vi "Install Libraries.vi"() -> ()   [LabVIEW 2021]
doc: "<b>_______________________________________________________________</b>\n** Author: Juan José Villacorta\n** LabVIEW wrapper for C library <b> wiringPi </b>,\n** https://github.com/WiringPi/WiringPi\n<b>_______________________________________________________________</b>\n\n\n/*\n * Install Helper\n ******************************************************************\n */"
uses:
  <vilib>/net/SSH/Client/OpenSSH/OpenSSH Client.lvclass
  C:/Program Files/National Instruments/LabVIEW 2026/vi.lib/net/SSH/Client/Generic/Generic Client.lvclass
  <vilib>/net/SSH/Client/Generic/Generic Client.lvclass/Generic Client.ctl
  <vilib>/net/SFTP/Session/Session.lvclass
  <vilib>/net/SFTP/NI_SFTP.lvlib
  <vilib>/net/SSH/NI_SSH.lvlib
  <vilib>/net/SFTP/API/Upload File.vi
  <vilib>/Utility/error.llb/DialogType.ctl
  <vilib>/net/SFTP/Connect (OpenSSH).vi
panel:
  in  "Close":bool
  in  "Install":bool
  out "Log":string caption="Error output"
  in  "password":string="raspberrypi"
  in  "User":string="pi"
  in  "Host":string="raspberrypi"
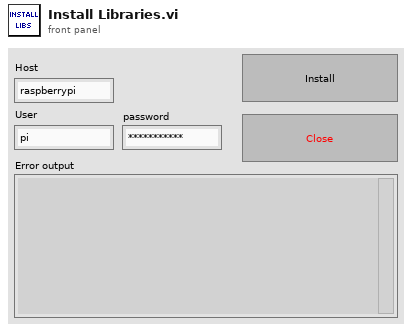
[diagram p1: front panel]
types:
  T1 = typedef "DialogType.ctl" = u16
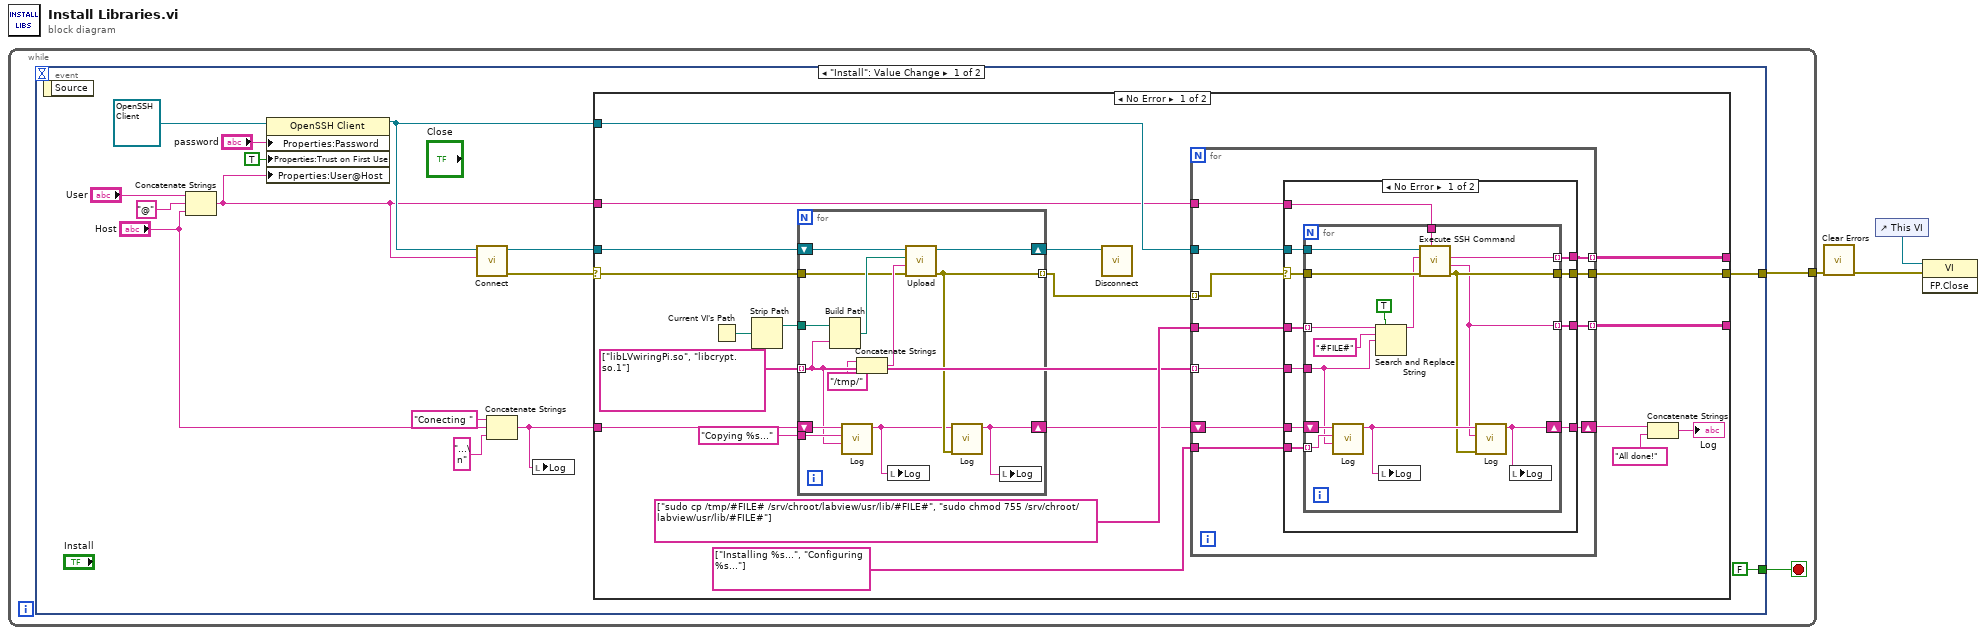
[diagram p0: block diagram]
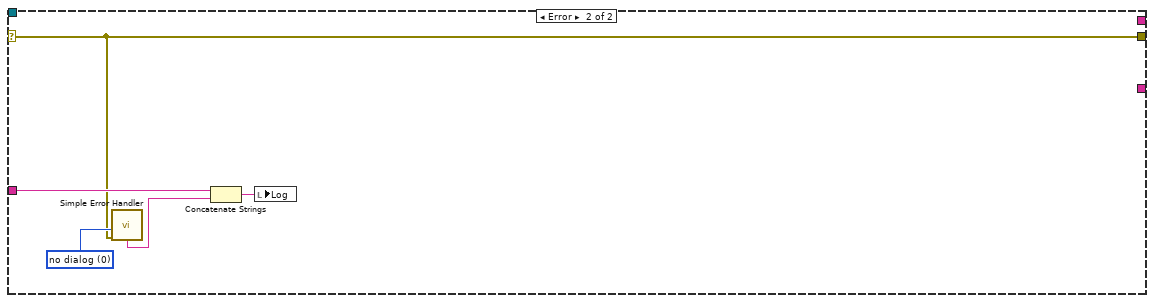
[diagram p3: hidden frame]
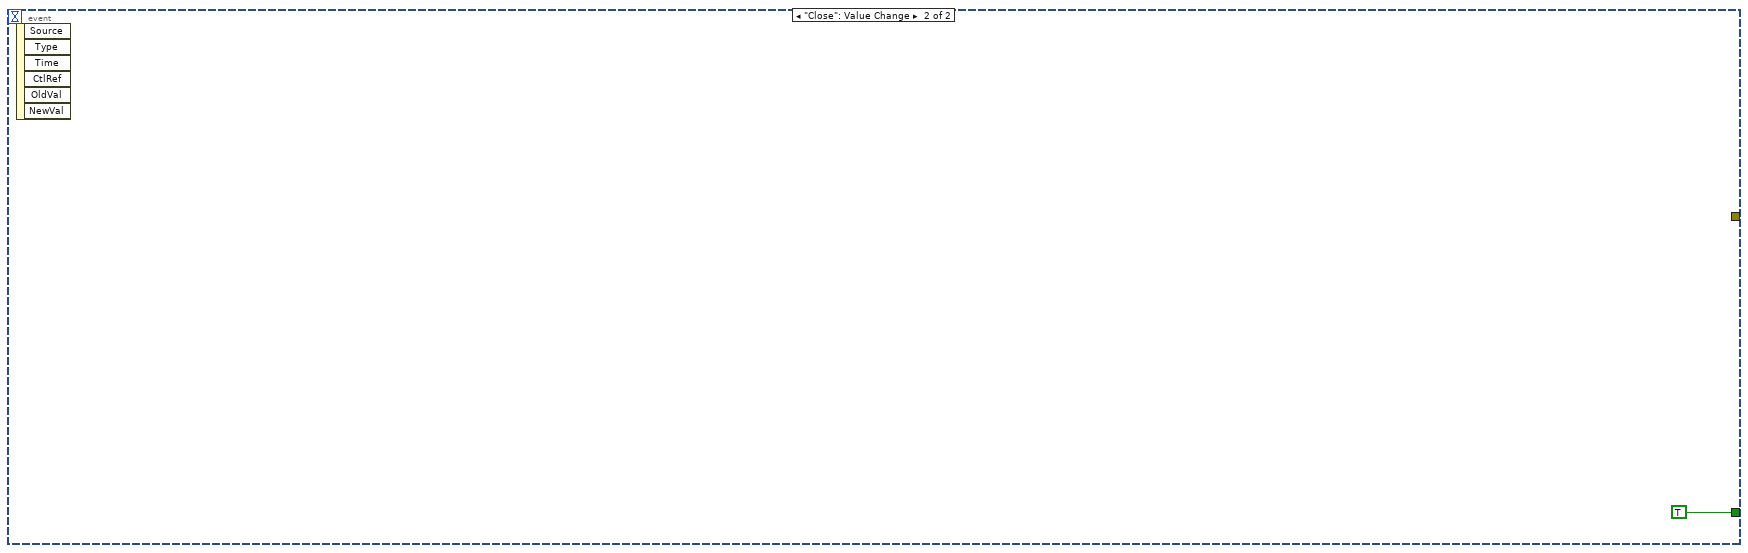
[diagram p4: hidden frame]
diagram:
  n1 = while {
    tunnel: [w5] -> w2
    stop <- w4 stop-if-true
    n2 = event shown="[0] \"Install\": Value Change" {
      selector: _ -> [_ _]
      dyn-events: _ -> [_ _]
      timeout: _ -> [_ _]
      tunnel: [w10 _] -> w5
      tunnel: [FALSE TRUE] -> w4
      event "Install": Value Change {
        n3 = event-data() -> ()  [unwired: 1 in, 1 out]
        n4 = Concatenate Strings("User", "@" ("string"), "Host") -> (w12:string)
        n5 = property class="OpenSSH Client"(reference=refnum<class "OpenSSH Client.lvclass"> refnum ("NI_SSH.lvlib:OpenSSH Client"), "Properties:Password"="password", "Properties:Trust on First Use"=TRUE ("trust on first use"), "Properties:User@Host"=w12) -> (reference out=w13:refnum<class "OpenSSH Client.lvclass">)  [unwired: 1 in, 1 out]
        n6 = call-poly <vilib>:"Connect.vi"("user@host"=w12, "client"=w13) -> ("error out"=w18:errorcluster, "session"=w19:refnum<class "Session.lvclass">)  [unwired: 8 in]
        n7 = Concatenate Strings("Conecting " ("string"), "Host", "...\n" ("string")) -> (w9:string)
        n8 = local write "Log"(w9) -> ()
        n9 = case shown="No Error" w18 {
          selector: w18 -> [w39 w92]
          tunnel: w19 -> [w40 _]
          tunnel: w13 -> [w35 _]
          tunnel: w12 -> [w34 _]
          tunnel: [w27 w92] -> w10
          tunnel: w9 -> [w23 w94]
          tunnel: [w22 _] -> _
          tunnel: [w21 _] -> _
          frame No Error {
            w32 = string[] ["libLVwiringPi.so", "libcrypt.so.1"] ("name or relative path")
            n10 = Current VI's Path() -> (path=w37:path)
            n11 = Strip Path(path=w37) -> (stripped path=w36:path)  [unwired: 1 out]
            n12 = for {
              tunnel: w36 -> [w88]
              tunnel: w32 -> [w82] mode=indexing
              shift-right: [w90] -> w38
              shift-left: w40 -> [w91]
              shift-right: [w79] -> w26
              shift-left: w23 -> [w84]
              tunnel: "Copying %s..." -> [w83]
              tunnel: w39 -> [w85]
              tunnel: [w81] -> w28 mode=indexing
              n13 = Build Path(base path=w88, name or relative path=w82) -> (appended path=w89:path)
              n14 = call "Log.vi"("Filename"=w82, "New Log"=w83, "Log In"=w84) -> ("Log out"=w80:string)  [unwired: 8 in]
              n15 = Concatenate Strings("/tmp/" ("string"), w82) -> (w87:string)
              n16 = local write "Log"(w80) -> ()
              n17 = call-poly <vilib>:"Upload.vi"("error in"=w85, "remote path"=w87, "local path"=w89, "session in"=w91) -> ("error out"=w81:errorcluster, "session out"=w90:refnum<class "Session.lvclass">)  [unwired: 6 in]
              n18 = call "Log.vi"("error in (no error)"=w81, "Log In"=w80) -> ("Log out"=w79:string)  [unwired: 9 in]
              n19 = local write "Log"(w79) -> ()
            }
            n20 = call-dynamic "Disconnect.vi"("session in"=w38) -> ()  [unwired: 7 in, 4 out]
            n21 = for {
              tunnel: w35 -> [w51]
              tunnel: w34 -> [w50]
              tunnel: string[] ["sudo cp /tmp/#FILE# /srv/chroot/labview/usr/lib/#FILE#", "sudo chmod 755 /srv/chroot/labview/usr/lib/#FILE#"] -> [w49]
              tunnel: w32 -> [w48] mode=indexing
              tunnel: w28 -> [w47] mode=indexing
              tunnel: [w46] -> w27
              shift-right: [w44] -> w24
              shift-left: w26 -> [w45]
              tunnel: string[] ["Installing %s...", "Configuring %s..."] -> [w43]
              tunnel: [w42] -> w22 mode=indexing
              tunnel: [w41] -> w21 mode=indexing
              n22 = case shown="No Error" w47 {
                selector: w47 -> [w58 _]
                tunnel: w51 -> [w62 _]
                tunnel: w50 -> [w61 _]
                tunnel: w49 -> [w60 _]
                tunnel: w48 -> [w59 _]
                tunnel: [w57 _] -> w46
                tunnel: w45 -> [w56 w78]
                tunnel: [w55 w78] -> w44
                tunnel: w43 -> [w54 _]
                tunnel: [w53 _] -> w42
                tunnel: [w52 _] -> w41
                frame No Error {
                  n23 = for {
                    tunnel: w62 -> [w77]
                    tunnel: w61 -> [w75]
                    tunnel: w60 -> [w67] mode=indexing
                    tunnel: w59 -> [w65]
                    tunnel: w58 -> [w76]
                    tunnel: [w66] -> w57
                    shift-right: [w70] -> w55
                    shift-left: w56 -> [w68]
                    tunnel: w54 -> [w69] mode=indexing
                    tunnel: [w64] -> w53 mode=indexing
                    tunnel: [w63] -> w52 mode=indexing
                    n24 = call "Log.vi"("Filename"=w65, "New Log"=w69, "Log In"=w68) -> ("Log out"=w71:string)  [unwired: 8 in]
                    n25 = Search and Replace String(replace all?=TRUE ("replace all? (F)"), input string=w67, search string="#FILE#", replace string=w65) -> (result string=w72:string)  [unwired: 4 in, 3 out]
                    n26 = local write "Log"(w71) -> ()
                    n27 = call <vilib>:"Execute SSH Command.vi"("user@host"=w75, "error in (no error)"=w76, "command line"=w72, "session in"=w77) -> ("error out"=w66:errorcluster, "standard error"=w63:string, "standard output"=w64:string)  [unwired: 3 in, 2 out]
                    n28 = call "Log.vi"("error in (no error)"=w66, "New Log"=w63, "Log In"=w71) -> ("Log out"=w70:string)  [unwired: 8 in]
                    n29 = local write "Log"(w70) -> ()
                  }
                }
                frame Error {
                }
              }
            }
            n30 = Concatenate Strings(w24, "All done!" ("string")) -> (→"Log":string)
          }
          frame Error {
            w96 = T1 0 items=["no dialog", "OK message", "continue or stop message", "OK message + warnings", "continue/stop + warnings"] ("type of dialog (OK msg:1)")
            n31 = call <vilib>:"Simple Error Handler.vi"("type of dialog (OK msg:1)"=w96, "error in (no error)"=w92) -> ("message"=w93:string)  [unwired: 3 in, 4 out]
            n32 = Concatenate Strings(w94, w93) -> (w95:string)
            n33 = local write "Log"(w95) -> ()
          }
        }
      }
      event "Close": Value Change {
        n34 = event-data() -> ()  [unwired: 1 in, 6 out]
      }
    }
  }
  n35 = call <vilib>:"Clear Errors.vi"("error in (no error)"=w2) -> ("error out"=w1:errorcluster)  [unwired: 5 in, 1 out]
  n36 = control-ref of="This VI"() -> (w3:refnum<vi>)
  n37 = invoke class="VI" method="FP.Close"(reference=w3, error in=w1) -> ()  [unwired: 1 in, 3 out]
